vi "Export Section Database Change to CSV.vi"(9 "Database Changes":T1 {"Missing"."Node Ref" format="%.0x"; "Changed"."Old"."Node Ref" format="%.0x"}, 10 "Section":string, 11 "Folder":path) -> (0 "error out":errorcluster)   [LabVIEW 2025, in "Protection and Counter Addon System Explorer.lvlib"]
uses:
  Protection and Counter Addon System Explorer.lvlib
  Types/Database Changes.ctl
  Types/Base Frame Info_NoVS.ctl
  Types/Signal Attributes.ctl
  Types/CAN Filter Type.ctl
  Types/Base Frame Info.ctl
  <vilib>/NI VeriStand/Custom Device API/Custom Device Item Ref.ctl
  Types/Related CAN Frames.ctl
  Types/Related CAN Frames No VS.ctl
  <vilib>/Utility/error.llb/Trim Whitespace One-Sided.vi
  <vilib>/NI VeriStand/Custom Device API/Custom Device API.lvlib
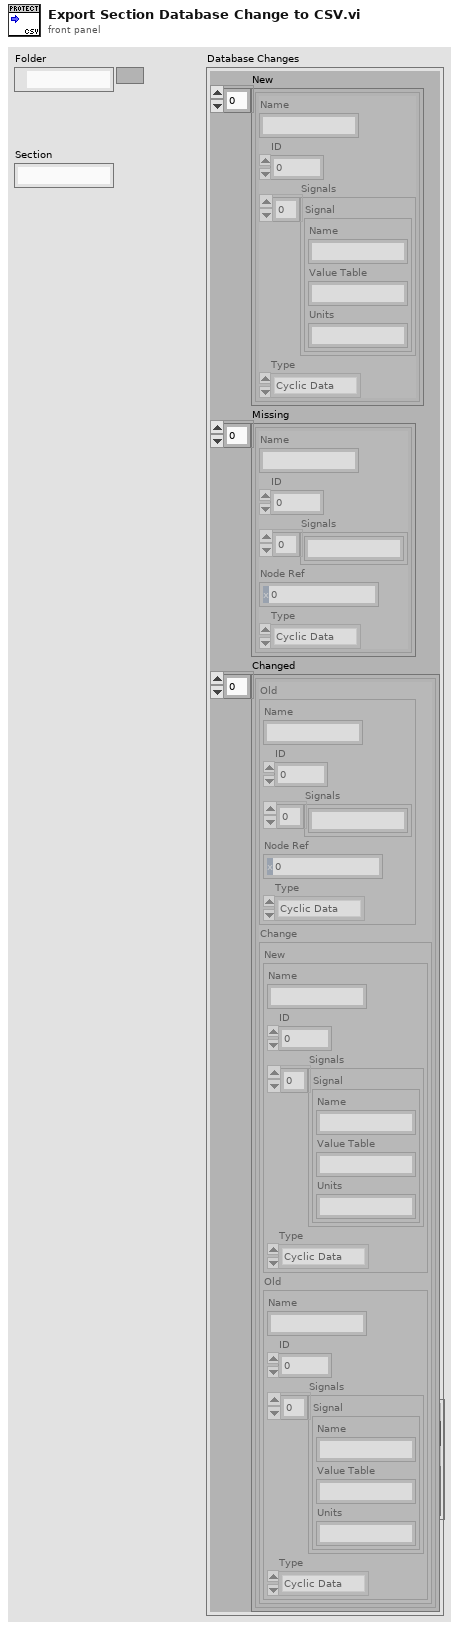
[diagram p1: front panel]
types:
  T1 = typedef "Protection and Counter Addon System Explorer.lvlib/Database Changes.ctl" = cluster{"New":T2[], "Missing":T5[], "Changed":T7[]}
  T2 = typedef "Protection and Counter Addon System Explorer.lvlib/Base Frame Info_NoVS.ctl" = cluster{"Name":string, "ID":u32, "Signals":T3[], "Type":T4}
  T3 = typedef "Protection and Counter Addon System Explorer.lvlib/Signal Attributes.ctl" = cluster{"Name":string, "Value Table":string, "Units":string}
  T4 = typedef "Protection and Counter Addon System Explorer.lvlib/CAN Filter Type.ctl" = enum16{"Cyclic Data", "Event Data", "Cyclic/Event", "All"}
  T5 = typedef "Protection and Counter Addon System Explorer.lvlib/Base Frame Info.ctl" = cluster{"Name":string, "ID":u32, "Signals":string[], "Node Ref":T6, "Type":T4}
  T6 = typedef "Custom Device API.lvlib/Custom Device Item Ref.ctl" = u64
  T7 = typedef "Protection and Counter Addon System Explorer.lvlib/Related CAN Frames.ctl" = cluster{"Old":T5, "Change":T8}
  T8 = typedef "Protection and Counter Addon System Explorer.lvlib/Related CAN Frames No VS.ctl" = cluster{"New":T2, "Old":T2}
  T9 = enum16{"open", "replace", "create", "open or create", "replace or create", "replace or create with confirmation"}
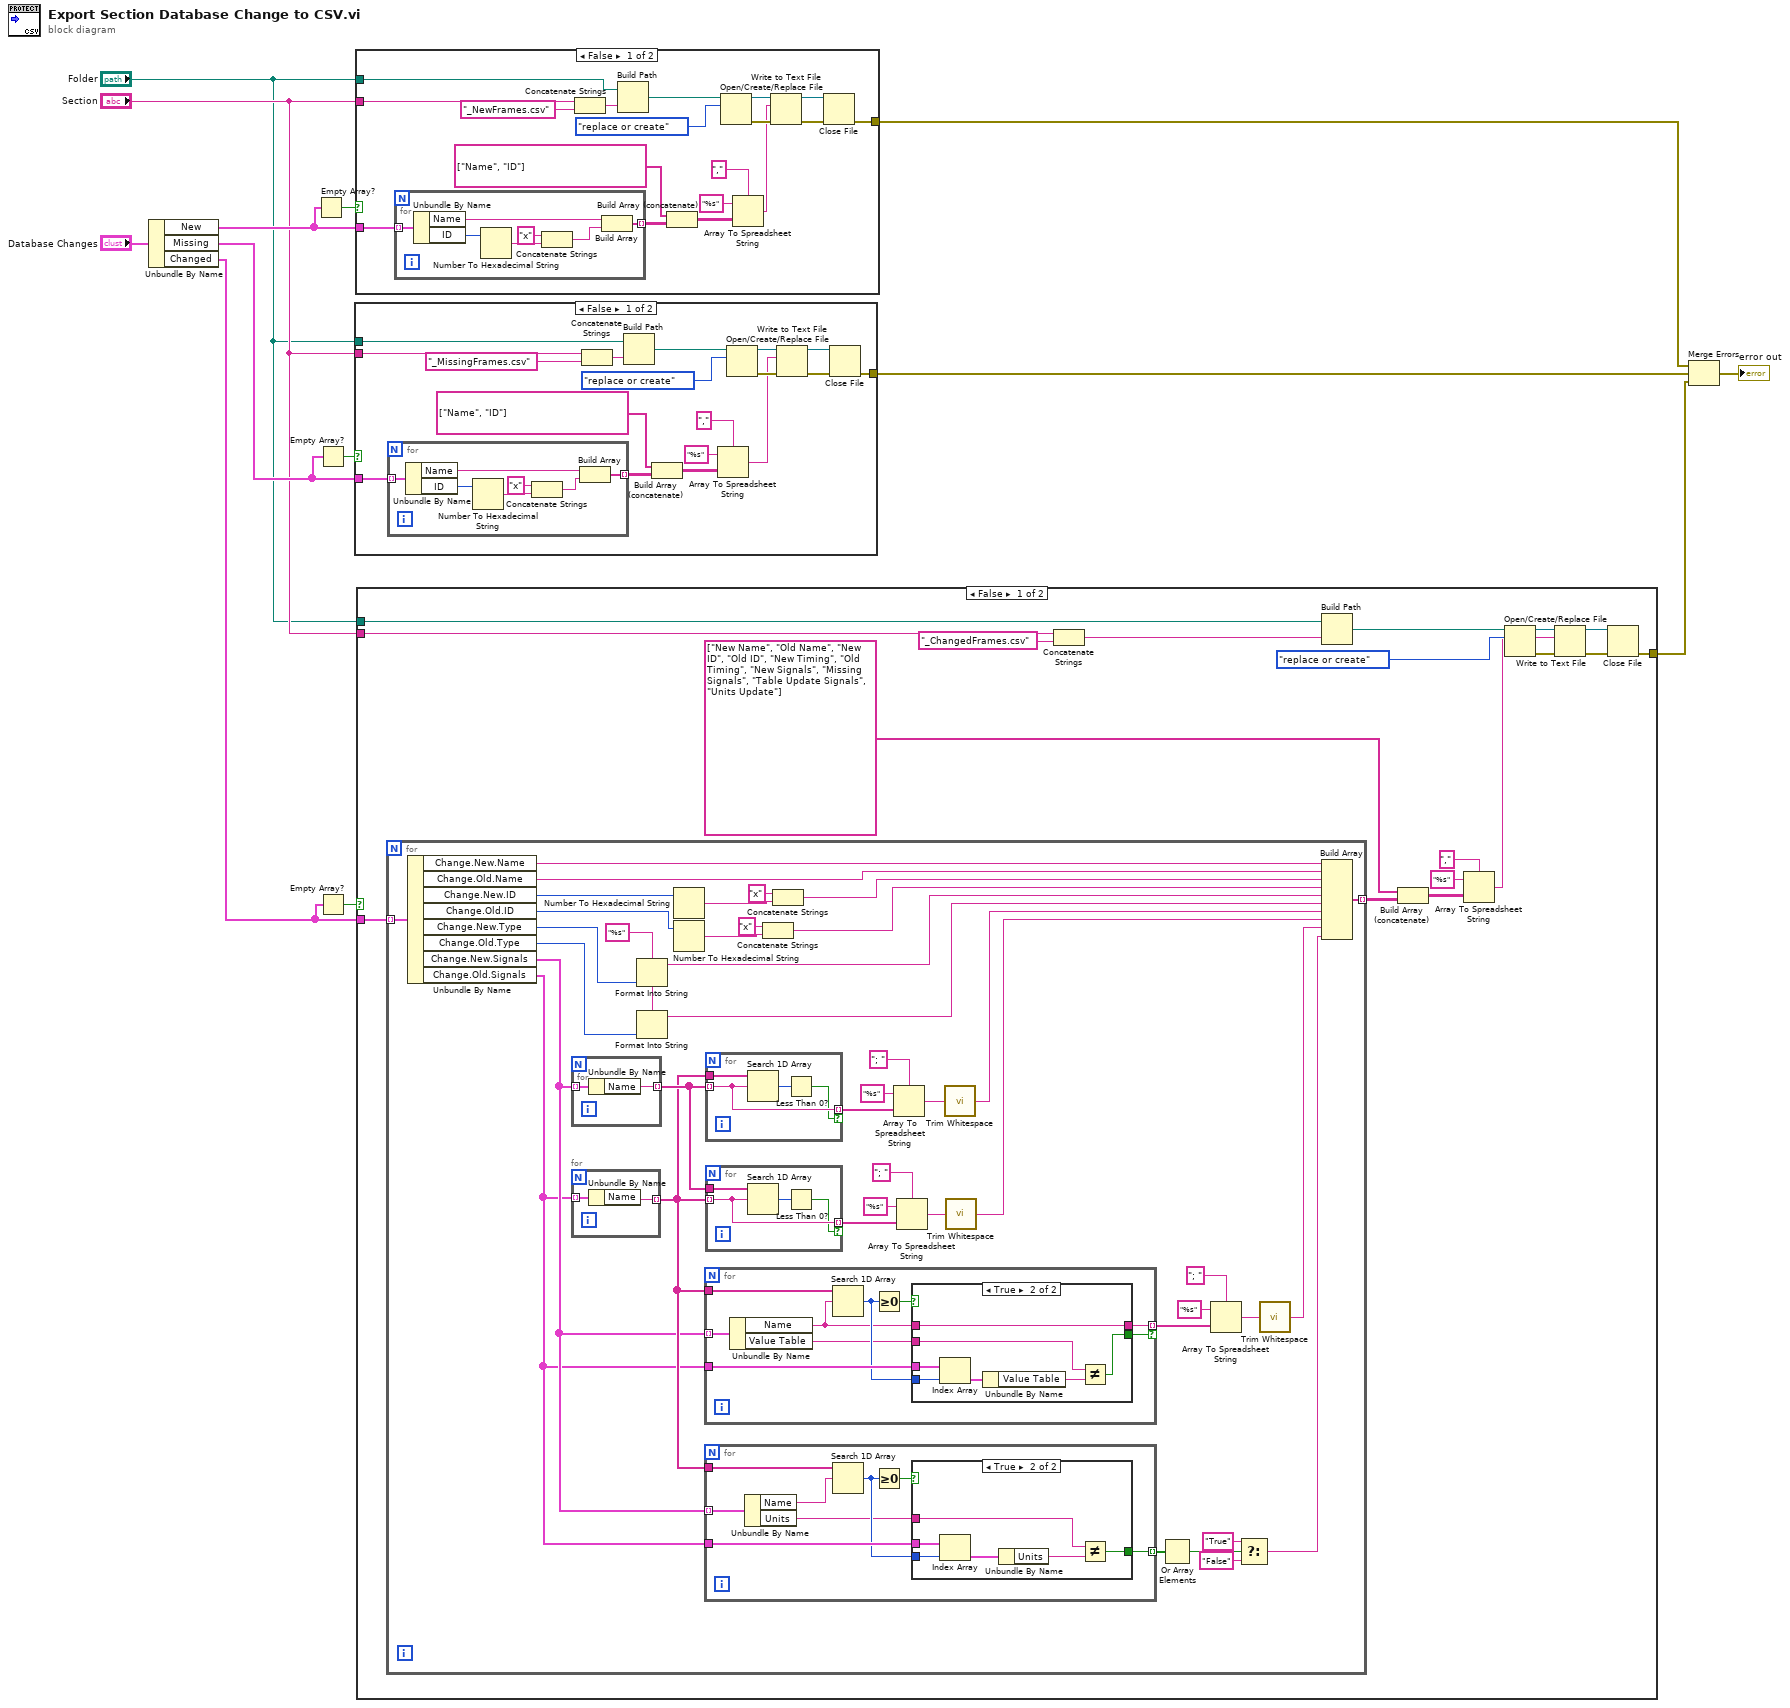
[diagram p0: block diagram]
diagram:
  n1 = Unbundle By Name("Database Changes") -> ("New"=w8:T2[], "Missing"=w11:T5[], "Changed"=w12:T7[])
  n2 = Empty Array?(array=w8) -> (empty?=w9:bool)
  n3 = Empty Array?(array=w11) -> (empty?=w10:bool)
  n4 = Empty Array?(array=w12) -> (empty?=w13:bool)
  n5 = case shown="False" w10 {
    tunnel: [w19 _] -> w3
    tunnel: "Folder" -> [w18 _]
    tunnel: "Section" -> [w15 _]
    tunnel: w11 -> [w14 _]
    frame False {
      n6 = for {
        tunnel: w14 -> [w38] mode=indexing
        tunnel: [w35] -> w28 mode=indexing
        n7 = Unbundle By Name(w38) -> ("Name"=w36:string, "ID"=w37:u32)
        n8 = Number To Hexadecimal String(2:w37) -> (0:w33:string)  [unwired: 1 in]
        n9 = Concatenate Strings("x" ("string"), w33) -> (w32:string)
        n10 = Build Array(w36, w32) -> (w35:string[])
      }
      n11 = Concatenate Strings(w15, "_MissingFrames.csv") -> (w16:string)
      n12 = Build Path(base path=w18, name or relative path=w16) -> (appended path=w20:path)
      n13 = Build Array (concatenate)(string[] ["Name", "ID"] ("appended array"), w28) -> (w31:string[][])
      n14 = Array To Spreadsheet String(delimiter (Tab)=",", array=w31, 3:"%s" ("format string")) -> (spreadsheet string=w21:string)
      n15 = Open/Create/Replace File(file path (use dialog)=w20, operation (0:open)=T9."replace or create") -> (refnum out=w25:refnum<file>, error out=w24:errorcluster)  [unwired: 4 in, 1 out]
      n16 = Write to Text File(file (use dialog)=w25, text=w21, error in=w24) -> (refnum out=w22:refnum<file>, error out=w23:errorcluster)  [unwired: 1 in, 1 out]
      n17 = Close File(refnum=w22, error in=w23) -> (error out=w19:errorcluster)  [unwired: 1 out]
    }
    frame True {
    }
  }
  n18 = case shown="False" w9 {
    tunnel: [w44 _] -> w2
    tunnel: "Folder" -> [w43 _]
    tunnel: "Section" -> [w40 _]
    tunnel: w8 -> [w39 _]
    frame False {
      n19 = for {
        tunnel: w39 -> [w63] mode=indexing
        tunnel: [w59] -> w53 mode=indexing
        n20 = Unbundle By Name(w63) -> ("Name"=w61:string, "ID"=w62:u32)
        n21 = Number To Hexadecimal String(2:w62) -> (0:w60:string)  [unwired: 1 in]
        n22 = Concatenate Strings("x" ("string"), w60) -> (w58:string)
        n23 = Build Array(w61, w58) -> (w59:string[])
      }
      n24 = Concatenate Strings(w40, "_NewFrames.csv") -> (w41:string)
      n25 = Build Path(base path=w43, name or relative path=w41) -> (appended path=w45:path)
      n26 = Build Array (concatenate)(string[] ["Name", "ID"] ("appended array"), w53) -> (w56:string[][])
      n27 = Open/Create/Replace File(file path (use dialog)=w45, operation (0:open)=T9."replace or create") -> (refnum out=w50:refnum<file>, error out=w49:errorcluster)  [unwired: 4 in, 1 out]
      n28 = Array To Spreadsheet String(delimiter (Tab)=",", array=w56, 3:"%s" ("format string")) -> (spreadsheet string=w46:string)
      n29 = Write to Text File(file (use dialog)=w50, text=w46, error in=w49) -> (refnum out=w47:refnum<file>, error out=w48:errorcluster)  [unwired: 1 in, 1 out]
      n30 = Close File(refnum=w47, error in=w48) -> (error out=w44:errorcluster)  [unwired: 1 out]
    }
    frame True {
    }
  }
  n31 = case shown="False" w13 {
    tunnel: w12 -> [w81 _]
    tunnel: [w68 _] -> w4
    tunnel: "Folder" -> [w67 _]
    tunnel: "Section" -> [w64 _]
    frame False {
      n32 = for {
        tunnel: w81 -> [w121] mode=indexing
        tunnel: [w117] -> w80 mode=indexing
        w104 = "%s" ("format string")
        n33 = Unbundle By Name(w121) -> ("Change.New.Name"=w122:string, "Change.Old.Name"=w119:string, "Change.New.ID"=w120:u32, "Change.Old.ID"=w118:u32, "Change.New.Type"=w105:T4, "Change.Old.Type"=w106:T4, "Change.New.Signals"=w88:T3[], "Change.Old.Signals"=w87:T3[])
        n34 = for {
          tunnel: w88 -> [w154] mode=indexing
          tunnel: [w153] -> w101 mode=indexing
          n35 = Unbundle By Name(w154) -> ("Name"=w153:string)
        }
        n36 = for {
          tunnel: w87 -> [w156] mode=indexing
          tunnel: [w155] -> w89 mode=indexing
          n37 = Unbundle By Name(w156) -> ("Name"=w155:string)
        }
        n38 = Format Into String(format string=w104, w105) -> (resulting string=w103:string)  [unwired: 2 in, 1 out]
        n39 = Format Into String(format string=w104, w106) -> (resulting string=w102:string)  [unwired: 2 in, 1 out]
        n40 = Number To Hexadecimal String(2:w120) -> (0:w93:string)  [unwired: 1 in]
        n41 = Number To Hexadecimal String(2:w118) -> (0:w91:string)  [unwired: 1 in]
        n42 = for {
          tunnel: w89 -> [w145]
          tunnel: w88 -> [w144] mode=indexing
          tunnel: w87 -> [w143]
          tunnel: [w139] -> w97 mode=indexing if=w137
          n43 = Unbundle By Name(w144) -> ("Name"=w138:string, "Value Table"=w140:string)
          n44 = Search 1D Array(1D array=w145, element=w138) -> (index of element=w142:i32)  [unwired: 1 in]
          n45 = Greater Or Equal To 0?(x=w142) -> (x >= 0?=w141:bool)
          n46 = case shown="True" w141 {
            tunnel: w143 -> [_ w152]
            tunnel: w142 -> [_ w151]
            tunnel: w140 -> [_ w148]
            tunnel: [_ w147] -> w139
            tunnel: w138 -> [_ w147]
            tunnel: [_ w146] -> w137
            frame False {
            }
            frame True {
              n47 = Index Array(array=w152, index=w151) -> (element=w150:T3)
              n48 = Unbundle By Name(w150) -> ("Value Table"=w149:string)
              n49 = Not Equal?(x=w148, y=w149) -> (x != y?=w146:bool)
            }
          }
        }
        n50 = for {
          tunnel: w89 -> [w130]
          tunnel: w88 -> [w129] mode=indexing
          tunnel: w87 -> [w128]
          tunnel: [w123] -> w86 mode=indexing
          n51 = Unbundle By Name(w129) -> ("Name"=w124:string, "Units"=w125:string)
          n52 = Search 1D Array(1D array=w130, element=w124) -> (index of element=w127:i32)  [unwired: 1 in]
          n53 = Greater Or Equal To 0?(x=w127) -> (x >= 0?=w126:bool)
          n54 = case shown="True" w126 {
            tunnel: w128 -> [_ w136]
            tunnel: w127 -> [_ w135]
            tunnel: w125 -> [_ w132]
            tunnel: [_ w131] -> w123
            frame False {
            }
            frame True {
              n55 = Index Array(array=w136, index=w135) -> (element=w134:T3)
              n56 = Unbundle By Name(w134) -> ("Units"=w133:string)
              n57 = Not Equal?(x=w132, y=w133) -> (x != y?=w131:bool)
            }
          }
        }
        n58 = for {
          tunnel: w89 -> [w160]
          tunnel: w101 -> [w158] mode=indexing
          tunnel: [w158] -> w112 mode=indexing if=w157
          n59 = Search 1D Array(1D array=w160, element=w158) -> (index of element=w159:i32)  [unwired: 1 in]
          n60 = Less Than 0?(x=w159) -> (x < 0?=w157:bool)
        }
        n61 = for {
          tunnel: w101 -> [w164]
          tunnel: w89 -> [w162] mode=indexing
          tunnel: [w162] -> w115 mode=indexing if=w161
          n62 = Search 1D Array(1D array=w164, element=w162) -> (index of element=w163:i32)  [unwired: 1 in]
          n63 = Less Than 0?(x=w163) -> (x < 0?=w161:bool)
        }
        n64 = Concatenate Strings("x" ("string"), w91) -> (w90:string)
        n65 = Concatenate Strings("x" ("string"), w93) -> (w92:string)
        n66 = Array To Spreadsheet String(delimiter (Tab)="; ", array=w112, 3:"%s" ("format string")) -> (spreadsheet string=w111:string)
        n67 = Array To Spreadsheet String(delimiter (Tab)="; ", array=w115, 3:"%s" ("format string")) -> (spreadsheet string=w116:string)
        n68 = call <vilib>:"Trim Whitespace.vi"("string"=w111) -> ("trimmed string"=w108:string)  [unwired: 1 in]
        n69 = call <vilib>:"Trim Whitespace.vi"("string"=w116) -> ("trimmed string"=w107:string)  [unwired: 1 in]
        n70 = Or Array Elements(Boolean array=w86) -> (logical OR=w85:bool)
        n71 = Array To Spreadsheet String(delimiter (Tab)="; ", array=w97, 3:"%s" ("format string")) -> (spreadsheet string=w100:string)
        n72 = Select(t="True", s=w85, f="False") -> (s? t:f=w82:string)
        n73 = call <vilib>:"Trim Whitespace.vi"("string"=w100) -> ("trimmed string"=w96:string)  [unwired: 1 in]
        n74 = Build Array(w122, w119, w92, w90, w103, w102, w108, w107, w96, w82) -> (w117:string[])
      }
      n75 = Concatenate Strings(w64, "_ChangedFrames.csv") -> (w65:string)
      n76 = Build Path(base path=w67, name or relative path=w65) -> (appended path=w69:path)
      n77 = Build Array (concatenate)(string[] ["New Name", "Old Name", "New ID", "Old ID", "New Timing", "Old Timing", "New Signals", "Missing Signals", "Table Update Signals", "Units Update"] ("appended array"), w80) -> (w78:string[][])
      n78 = Array To Spreadsheet String(delimiter (Tab)=",", array=w78, 3:"%s" ("format string")) -> (spreadsheet string=w70:string)
      n79 = Open/Create/Replace File(file path (use dialog)=w69, operation (0:open)=T9."replace or create") -> (refnum out=w74:refnum<file>, error out=w73:errorcluster)  [unwired: 4 in, 1 out]
      n80 = Write to Text File(file (use dialog)=w74, text=w70, error in=w73) -> (refnum out=w71:refnum<file>, error out=w72:errorcluster)  [unwired: 1 in, 1 out]
      n81 = Close File(refnum=w71, error in=w72) -> (error out=w68:errorcluster)  [unwired: 1 out]
    }
    frame True {
    }
  }
  n82 = Merge Errors(w2, w3, w4) -> (→"error out":errorcluster)
